vi "List Control Elements.vi"(10 "path":string, 11 "control":refnum<vi>) -> (2 "element paths":string[](array[string]), 3 "element controls":refnum<vi>[](array[refnum]))   [LabVIEW 2020, in "MCP Server.lvlib"]
doc: "Lists the elements of a front panel control together with the JSON path of each element in the control's JSON Schema, for Add Control Details To Schema.vi. A cluster gives its elements under path.properties.<label>, an array its element under path.items (once per dimension). Any other control has no elements."
uses:
  MCP Server.lvlib
  699e7f21-2791-4bce-b0e1-8e9ee76c4c3a.vi
  <vilib>/JDP Science/JSONtext/Variant to JSON Text.vi
  <vilib>/JDP Science/JSONtext/LVClass Serializer/JSONtext LVClass Serializer.lvclass
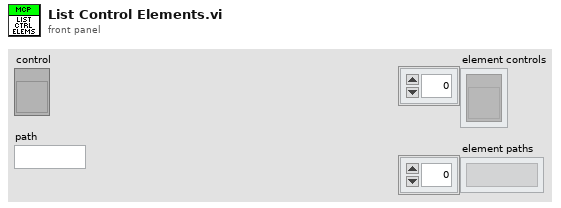
[diagram p1: front panel]
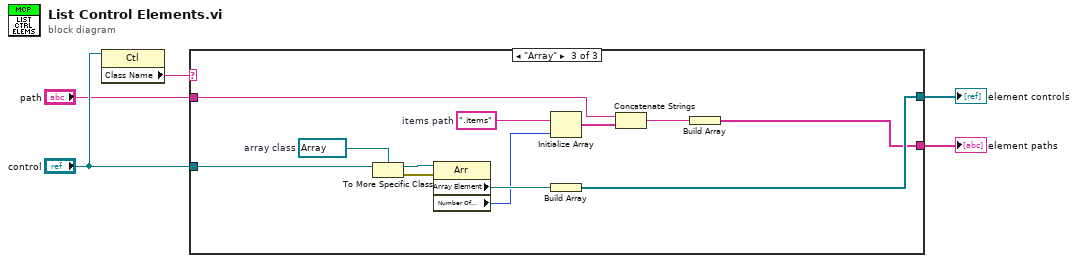
[diagram p0: block diagram]
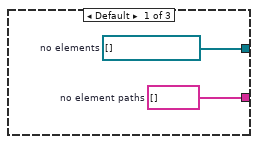
[diagram p2: hidden frame]
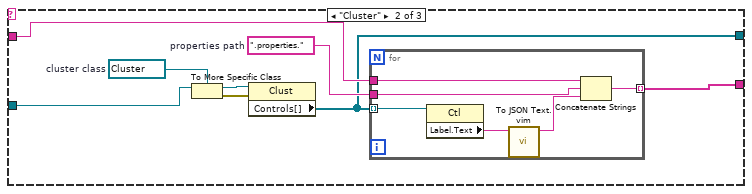
[diagram p3: hidden frame]
diagram:
  n1 = property class="Ctl"(reference="control") -> ("Class Name"=w3:string)  [unwired: 1 in, 2 out]
  n2 = case shown="\"Array\"" w3 {
    tunnel: "control" -> [_ w15 w33]
    tunnel: "path" -> [_ w11 w26]
    tunnel: [w7 w9 w23] -> w2
    tunnel: [w6 w8 w22] -> w1
    frame Default {
      w6 = string[] []  # no element paths
      w7 = refnum<vi>[] []  # no elements
    }
    frame "Cluster" {
      w10 = ".properties."  # properties path
      w14 = refnum<vi> refnum  # cluster class
      n3 = To More Specific Class(target class=w14, reference=w15) -> (specific class reference=w13:refnum<vi>, error out=w12:errorcluster)  [unwired: 1 in]
      n4 = property class="Clust"(reference=w13, error in=w12) -> ("Controls[]"=w9:refnum<vi>[])  [unwired: 2 out]
      n5 = for {
        tunnel: w9 -> [w21] mode=indexing
        tunnel: w11 -> [w19]
        tunnel: w10 -> [w18]
        tunnel: [w16] -> w8 mode=indexing
        n6 = property class="Ctl"(reference=w21) -> ("Label.Text"=w20:string)  [unwired: 1 in, 2 out]
        n7 = call "To JSON Text.vim"("Anything"=w20) -> ("<JSON>"=w17:string)  [unwired: 9 in, 1 out]
        n8 = Concatenate Strings(w19, w18, w17) -> (w16:string)
      }
    }
    frame "Array" {
      w28 = ".items"  # items path
      w32 = refnum<vi> refnum  # array class
      n9 = To More Specific Class(target class=w32, reference=w33) -> (specific class reference=w31:refnum<vi>, error out=w30:errorcluster)  [unwired: 1 in]
      n10 = property class="Arr"(reference=w31, error in=w30) -> ("Array Element"=w29:refnum<vi>, "Number Of Dimensions"=w27:u32)  [unwired: 2 out]
      n11 = Initialize Array(w28, w27) -> (w25:string[])
      n12 = Build Array(w29) -> (w23:refnum<vi>[])
      n13 = Concatenate Strings(w26, w25) -> (w24:string)
      n14 = Build Array(w24) -> (w22:string[])
    }
  }
  "element controls" <- w2
  "element paths" <- w1
